vi "Write Test Info.vi"(8 "error in (no error)":errorcluster, 10 "Test Info":T1={"General"={"Operator"="JLee"}}, 11 "CSL configuration":refnum<class "CSL configuration.lvclass">) -> (0 "error out":errorcluster, 3 "CSL configuration out":refnum<class "CSL configuration.lvclass">)   [LabVIEW 2025, in "CSL.lvlib" / "CSL configuration.lvclass"]
uses:
  CSL configuration.lvclass
  Test Info.ctl
  CSL configuration.lvclass/CSL configuration.ctl
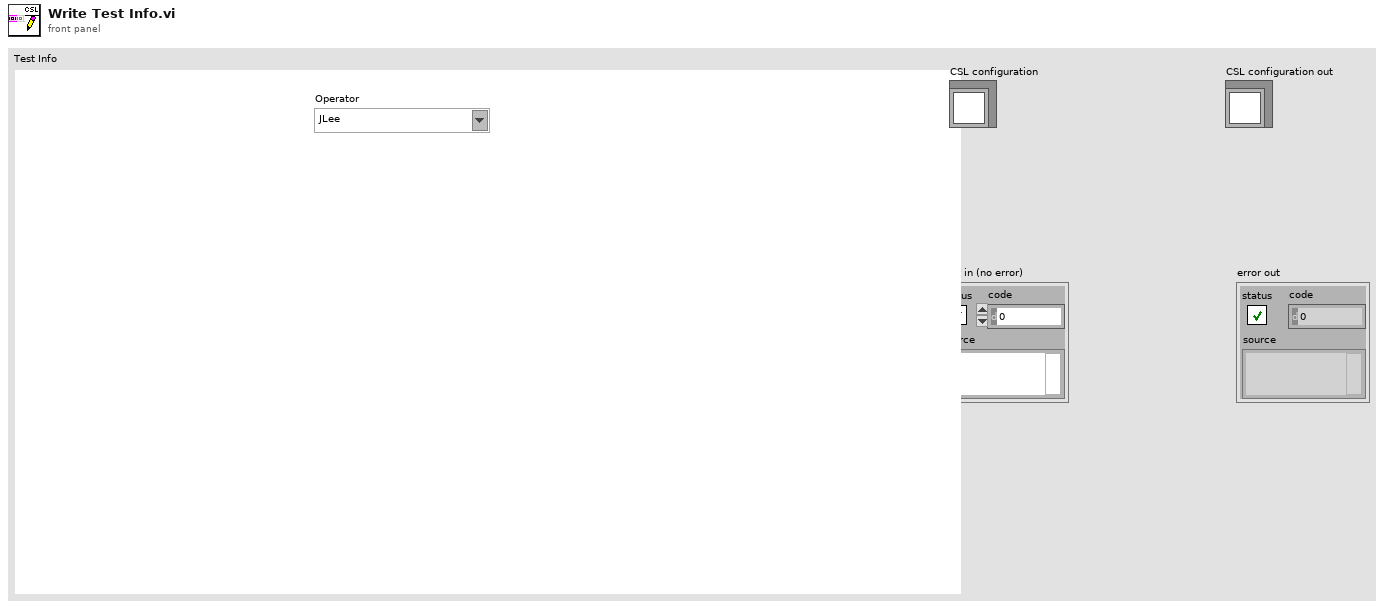
[diagram p1: front panel]
types:
  T1 = typedef "CSL.lvlib/CSL configuration.lvclass/Test Info.ctl" = cluster{"General":cluster{"Operator":string}}
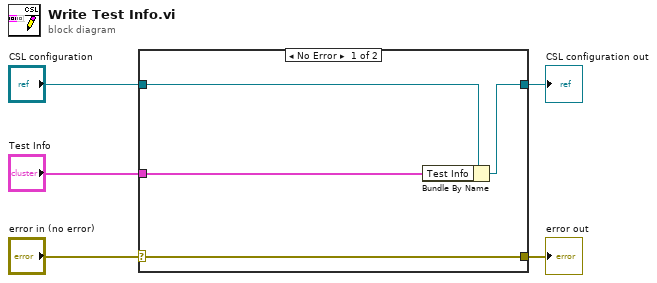
[diagram p0: block diagram]
diagram:
  n1 = case shown="No Error" "error in (no error)" {
    selector: "error in (no error)" -> [w9 w10]
    tunnel: [w9 w10] -> w4
    tunnel: [w7 w11] -> w1
    tunnel: "CSL configuration" -> [w8 w11]
    tunnel: "Test Info" -> [w6 _]
    frame No Error {
      n2 = Bundle By Name(cluster=w8, "Test Info"=w6) -> (w7:refnum<class "CSL configuration.lvclass">)
    }
    frame Error {
    }
  }
  "error out" <- w4
  "CSL configuration out" <- w1
